vi "set Swept SA - Sweep Count.vi"(8 "error in (no error)":errorcluster, 10 "Sweep Count":u32, 11 "Keysight 9020A in":refnum<class "Keysight 9020A.lvclass">) -> (0 "error out":errorcluster, 3 "Keysight 9020A out":refnum<class "Keysight 9020A.lvclass">)   [LabVIEW 2023, in "Spectrum Analyzer.lvlib" / "Keysight 9020A.lvclass"]
doc: "This command defines the number of sweeps started with single sweep, which are\nused for calculating the average or maximum value. If the values 0 or 1 are set, one\nsweep is performed.\n\n* For FSV-40\n1) Parameters:\n<NumberSweeps> 0 to 32767\n *RST: 0 (GSM: 200, PHN:1)\nExample: SWE:COUN 64\n Sets the number of sweeps to 64.\n INIT:CONT OFF\n Switches to single sweep mode.\n INIT;*WAI\n Starts a sweep and waits for its end."
uses:
  Keysight 9020A.lvclass
  Keysight 9020A.lvclass/Keysight 9020A.ctl
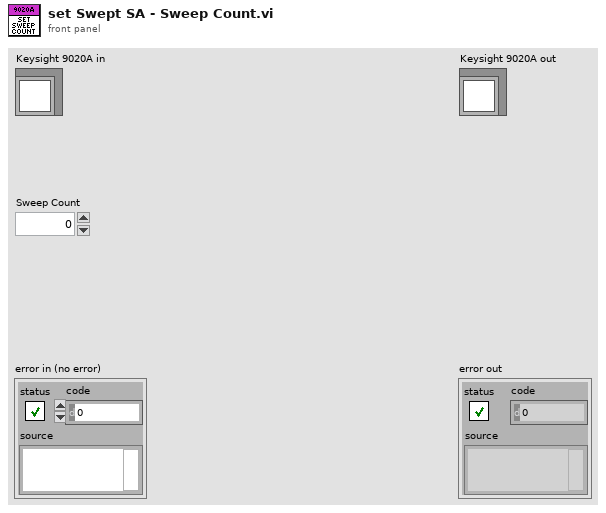
[diagram p1: front panel]
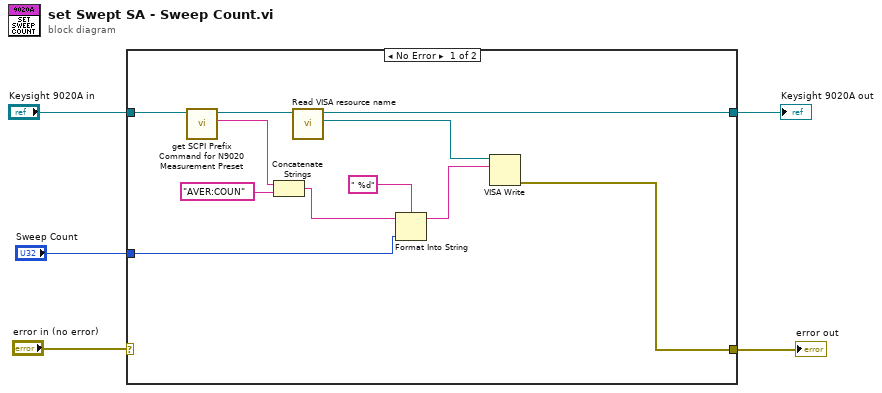
[diagram p0: block diagram]
diagram:
  n1 = case shown="No Error" "error in (no error)" {
    selector: "error in (no error)" -> [_ w17]
    tunnel: "Keysight 9020A in" -> [w10 w18]
    tunnel: [w16 w18] -> w4
    tunnel: [w12 w17] -> w2
    tunnel: "Sweep Count" -> [w11 _]
    frame No Error {
      n2 = call "get SCPI Prefix Command for N9020 Measurement Preset.vi"("Keysight 9020A in"=w10) -> ("SCPI Prefix Command"=w7:string, "Keysight 9020A out"=w9:refnum<class "Keysight 9020A.lvclass">)  [unwired: 8 in, 1 out]
      n3 = Concatenate Strings(w7, "AVER:COUN") -> (w6:string)
      n4 = call "Read VISA resource name.vi"("Keysight 9020A in"=w9) -> ("VISA resource name"=w14:refnum<visa-resource-name>, "Keysight 9020A out"=w16:refnum<class "Keysight 9020A.lvclass">)  [unwired: 8 in, 1 out]
      n5 = Format Into String(format string=" %d", initial string=w6, w11) -> (resulting string=w13:string)  [unwired: 1 in, 1 out]
      n6 = VISA Write(VISA resource name=w14, write buffer=w13) -> (error out=w12:errorcluster)  [unwired: 1 in, 2 out]
    }
    frame Error {
    }
  }
  "error out" <- w2
  "Keysight 9020A out" <- w4
